vi "nominal open.vi"(7 "Timeout ms (-1: infinite)":i32=-1, 9 "Workspace (tenant default)":string, 10 "Base URL":string="https://api.gov.nominal.io/api", 11 "API key":string) -> (0 "error out":errorcluster, 3 "connection":refnum<class "Nominal Client.lvclass">)   [LabVIEW 2020, in "nominal core steps.lvlib"]
doc: "Opens a connection to Nominal.\n\nTo get the required inputs, review getting started material in the docs or go straight to Nominal settings. In the settings, go to the \"API keys\" page to get your API key, workspace RID, and base URL."
uses:
  nominal core steps.lvlib
  <vilib>/Nominal/Nominal IO Client/lv_src/Nominal Client/Nominal Client.lvclass
  <vilib>/Nominal/Nominal IO Client/lv_src/Nominal Client/Nominal Client.lvclass/Nominal Client.ctl
  <vilib>/Nominal/Nominal IO Client/lv_src/nominal types/workspace/workspace.lvclass/workspace.ctl
  5fae3aaa-2d6c-40fa-a575-248e876d1dec.vi
  <vilib>/Nominal/Nominal IO Client/lv_src/Nominal Client/private_data.set.vi
  5fae3aaa-2d6c-40fa-a575-248e876d1dec.vi/8284acbc-2d4d-4b18-b492-8ff51a6e7e10.vi
  <vilib>/Nominal/Nominal IO Client/lv_src/Nominal Client/Palette Items/destroy.vi
  <vilib>/Nominal/Nominal IO Client/lv_src/nominal types/workspace/id.get.vi
  <vilib>/Nominal/Nominal IO Client/lv_src/nominal types/workspace/rid.get.vi
  <vilib>/AdvancedString/1D String Array to Delimited String.vi
  <vilib>/Nominal/Nominal IO Client/lv_src/Nominal Client/workspace.set.vi
  <vilib>/Utility/file.llb/Application Directory.vi
  <vilib>/Utility/error.llb/Error Cluster From Error Code.vi
  <vilib>/Nominal/Nominal IO Client/lv_src/Nominal Client/format endpoint termination.vi
  <vilib>/Nominal/Nominal IO Client/submodules/reqwest-labview/lv-src/reqwest/create.vi
  <vilib>/Nominal/Nominal IO Client/lv_src/Nominal Client/workspace_cache.get_from_rid.vi
  <vilib>/Nominal/Nominal IO Client/lv_src/Nominal Client/workspace_cache.get.vi
  <vilib>/Nominal/Nominal IO Client/lv_src/Nominal Client/Palette Items/who_am_i.vi
  <vilib>/Nominal/Nominal IO Client/submodules/reqwest-labview/lv-src/reqwest/destroy.vi
  <vilib>/Nominal/Nominal IO Client/lv_src/User/User.lvclass
  <vilib>/Nominal/Nominal IO Client/lv_src/nominal types/workspace/workspace.lvclass
  <vilib>/Nominal/Nominal IO Client/submodules/reqwest-labview/lv-src/reqwest/reqwest.lvclass
  <vilib>/Nominal/Nominal IO Client/submodules/reqwest-labview/lv-src/reqwest/header.ctl
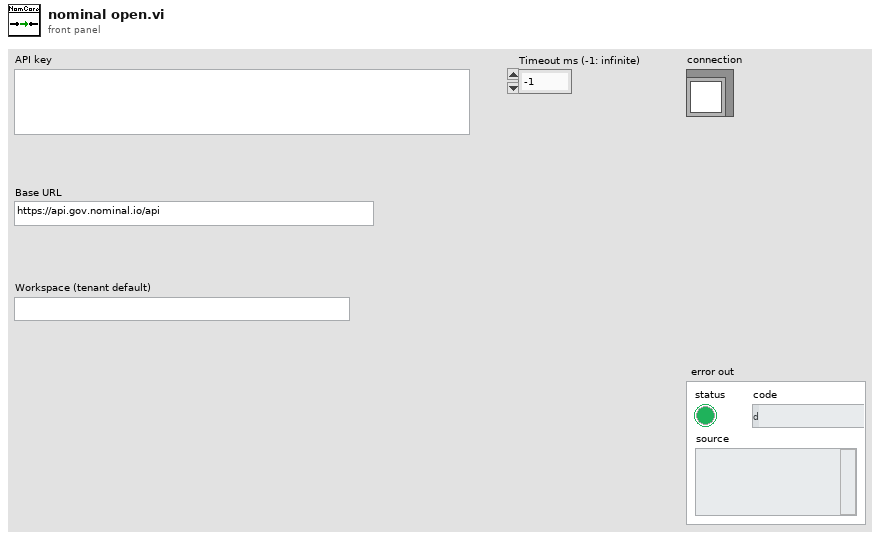
[diagram p1: front panel]
types:
  T1 = typedef "reqwest.lvclass/header.ctl" = cluster{"header":string, "value":string}
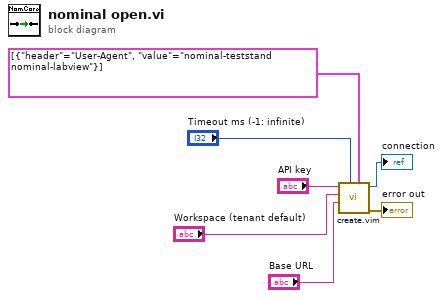
[diagram p0: block diagram]
diagram:
  n1 = call "create.vim"("Default Headers ([JSON])"=T1[] [{"header"="User-Agent", "value"="nominal-teststand nominal-labview"}], "Timeout ms (-1: infinite)"="Timeout ms (-1: infinite)", "Base URL"="Base URL", "Workspace"="Workspace (tenant default)", "API Token (string or path)"="API key") -> ("error out"=→"error out":errorcluster, "Nominal Client"=→"connection":refnum<class "Nominal Client.lvclass">)  [unwired: 4 in, 1 out]
